vi "API Proxy - Open and Run All Tests.vi"() -> ()   [LabVIEW 2017]
panel:
  in  "application reference":refnum<vi>
  out "error out":errorcluster
  in  "error in (no error)":errorcluster
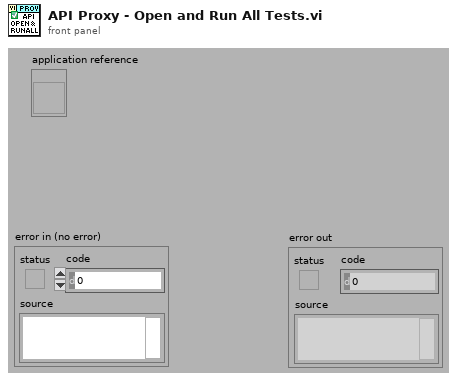
[diagram p1: front panel]
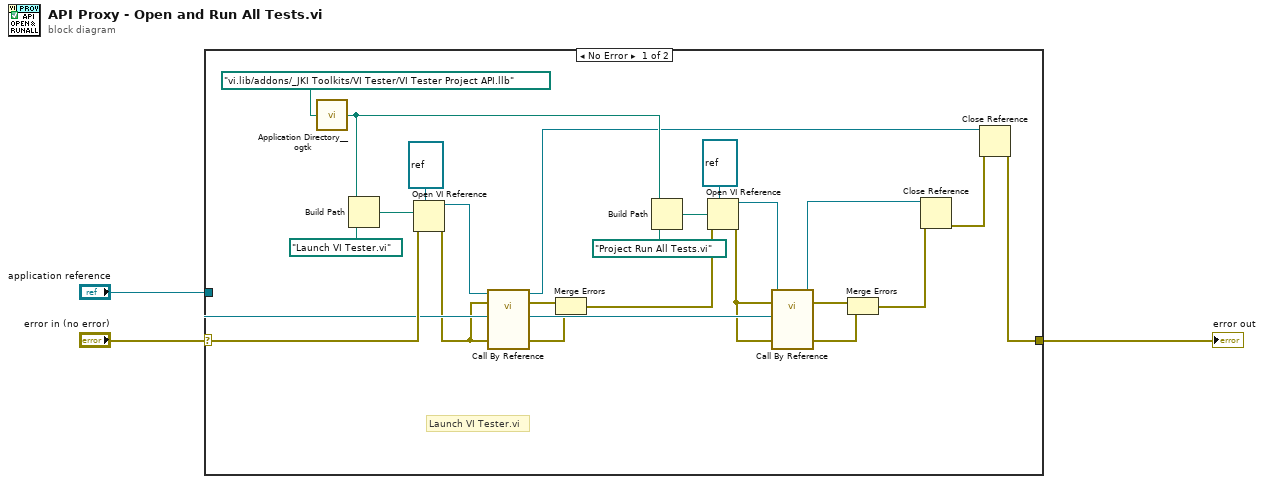
[diagram p0: block diagram]
diagram:
  n1 = case shown="No Error" "error in (no error)" {
    selector: "error in (no error)" -> [w25 w29]
    tunnel: [w4 w29] -> w2
    tunnel: "application reference" -> [w23 _]
    frame No Error {
      # "Launch VI Tester.vi"
      n2 = call <userlib>:"Application Directory__ogtk.vi"("Relative path (.)"=path "vi.lib/addons/_JKI Toolkits/VI Tester/VI Tester Project API.llb") -> ("Application Directory (+ Relative)"=w16:path)
      n3 = Build Path(base path=w16, name or relative path=path "Launch VI Tester.vi") -> (appended path=w26:path)
      n4 = Open VI Reference(type specifier VI Refnum (for type only)=refnum<vi> refnum, vi path=w26, error in (no error)=w25) -> (vi reference=w15:refnum<vi>, error out=w22:errorcluster)  [unwired: 3 in]
      n5 = call-by-ref "?"(reference=w15, error in=w22, 8:"error in (no error)"=w22, "application reference"=w23) -> (reference out=w7:refnum<vi>, error out=w14:errorcluster, 0:"error out"=w11:errorcluster, "VI Tester Ref"=w19:refnum<vi>)  [unwired: 7 in, 1 out]
      n6 = Merge Errors(w14, w11) -> (w12:errorcluster)
      n7 = Build Path(base path=w16, name or relative path=path "Project Run All Tests.vi") -> (appended path=w18:path)
      n8 = Open VI Reference(type specifier VI Refnum (for type only)=refnum<vi> refnum, vi path=w18, error in (no error)=w12) -> (vi reference=w20:refnum<vi>, error out=w13:errorcluster)  [unwired: 3 in]
      n9 = call-by-ref "?"(reference=w20, error in=w13, 8:"error in (no error)"=w13, "VI Tester reference"=w19) -> (reference out=w8:refnum<vi>, error out=w10:errorcluster, 0:"error out"=w9:errorcluster)  [unwired: 9 in]
      n10 = Merge Errors(w10, w9) -> (w5:errorcluster)
      n11 = Close Reference(reference=w8, error in (no error)=w5) -> (error out=w6:errorcluster)
      n12 = Close Reference(reference=w7, error in (no error)=w6) -> (error out=w4:errorcluster)
    }
    frame Error {
    }
  }
  "error out" <- w2
